vi "export labview dosctrings.vi"() -> ()   [LabVIEW 2020]
panel:
  out "error out":errorcluster
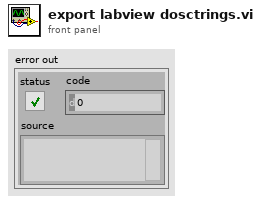
[diagram p1: front panel]
types:
  T1 = enum32{"invalid VI type", "Standard VI", "Control VI", "Global VI", "Polymorphic VI", "Configuration VI", "SubSystem", "Facade VI", "Method VI", "Statechart Diagram VI"}
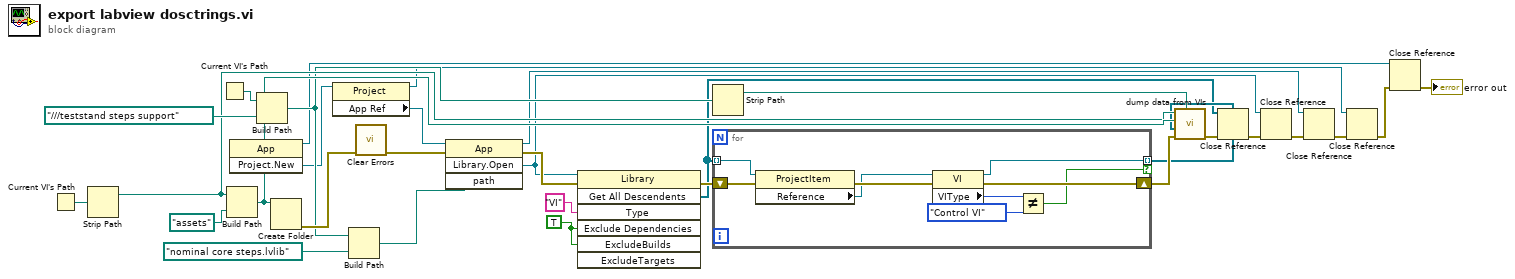
[diagram p0: block diagram]
diagram:
  w2 = TRUE ("ExcludeDependencies")
  n1 = Current VI's Path() -> (path=w30:path)
  n2 = Strip Path(path=w30) -> (stripped path=w26:path)  [unwired: 1 out]
  n3 = Current VI's Path() -> (path=w24:path)
  n4 = Build Path(base path=w26, name or relative path=path "assets") -> (appended path=w27:path)
  n5 = invoke class="App" method="Project.New"() -> (reference out=w13:refnum<vi>, "Project:New"=w20:refnum<vi>)  [unwired: 3 in, 1 out]
  n6 = Build Path(base path=w24, name or relative path=path "../../../teststand steps support") -> (appended path=w22:path)
  n7 = Create Folder(path (use dialog)=w27) -> (error out=w28:errorcluster)  [unwired: 2 in, 2 out]
  n8 = property class="Project"(reference=w20) -> (reference out=w12:refnum<vi>, "App Ref"=w19:refnum<vi>)  [unwired: 1 in, 1 out]
  n9 = Build Path(base path=w22, name or relative path=path "nominal core steps.lvlib") -> (appended path=w17:path)
  n10 = call <vilib>:"Clear Errors.vi"("error in (no error)"=w28) -> ("error out"=w18:errorcluster)  [unwired: 5 in, 1 out]
  n11 = invoke class="App" method="Library.Open"(reference=w19, error in=w18, "path"=w17) -> (reference out=w11:refnum<vi>, error out=w9:errorcluster, "Open Library"=w8:refnum<vi>)  [unwired: 1 in, 1 out]
  n12 = invoke class="Library" method="Get All Descendents"(reference=w8, error in=w9, "Type"="VI", "Exclude Dependencies"=w2, "ExcludeBuilds"=w2) -> (error out=w7:errorcluster, "All Descendents"=w1:refnum<vi>[])  [unwired: 2 in, 5 out]
  n13 = Strip Path(path=w22) -> (stripped path=w25:path)  [unwired: 1 out]
  n14 = for {
    shift-right: [w37] -> w5
    shift-left: w7 -> [w40]
    tunnel: w1 -> [w38] mode=indexing
    tunnel: [w35] -> w3 mode=indexing if=w32
    n15 = property class="ProjectItem"(reference=w38, error in=w40) -> (error out=w39:errorcluster, "Reference"=w36:refnum<vi>)  [unwired: 1 out]
    n16 = property class="VI"(reference=w36, error in=w39) -> (reference out=w35:refnum<vi>, error out=w37:errorcluster, "VIType"=w34:T1)
    n17 = Not Equal?(x=w34, y=T1."Control VI") -> (x != y?=w32:bool)
  }
  n18 = call "dump data from VIs.vi"("base"=w25, "error in (no error)"=w5, "vi references"=w3, "assets"=w27, "docs folder"=w26) -> ("error out"=w23:errorcluster)  [unwired: 6 in]
  n19 = Close Reference(reference=w1, error in (no error)=w23) -> (error out=w4:errorcluster)
  n20 = Close Reference(reference=w8, error in (no error)=w4) -> (error out=w10:errorcluster)
  n21 = Close Reference(reference=w11, error in (no error)=w10) -> (error out=w16:errorcluster)
  n22 = Close Reference(reference=w12, error in (no error)=w16) -> (error out=w14:errorcluster)
  n23 = Close Reference(reference=w13, error in (no error)=w14) -> (error out=→"error out":errorcluster)
